vi "TestGeneralSyntax.vi"(8 "error in (no error)":errorcluster) -> (0 "error out":errorcluster)   [LabVIEW 2019]
uses:
  <vilib>/addons/_JKI Toolkits/Caraya/classes/Test/Test.lvclass
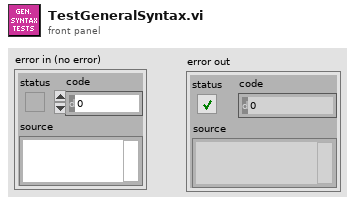
[diagram p1: front panel]
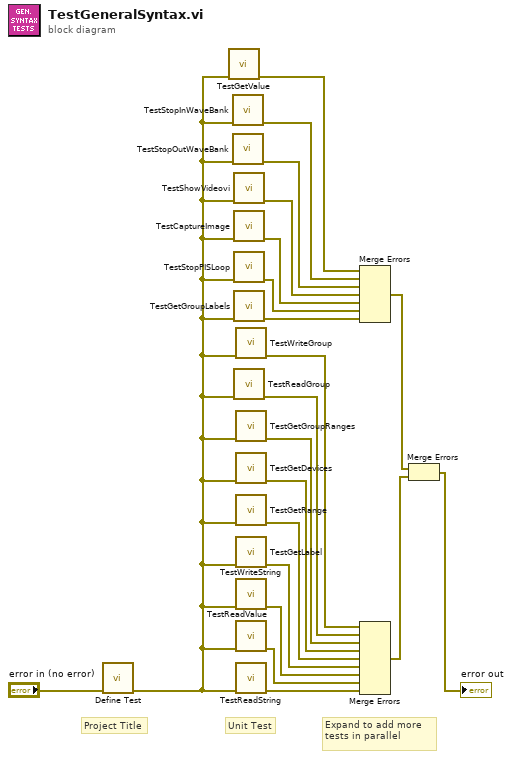
[diagram p0: block diagram]
diagram:
  # "Expand to add more tests in parallel"
  # "Unit Test"
  # "Project Title"
  n1 = call <vilib>:"Define Test.vi"("error in (no error)"="error in (no error)") -> ("error out"=w1:errorcluster)  [unwired: 10 in]
  n2 = call "TestGetValue.vi"("error in (no error)"=w1) -> ("error out"=w2:errorcluster)  [unwired: 10 in]
  n3 = call "TestStopInWaveBank.vi"("error in (no error)"=w1) -> ("error out"=w3:errorcluster)  [unwired: 10 in]
  n4 = call "TestStopOutWaveBank.vi"("error in (no error)"=w1) -> ("error out"=w4:errorcluster)  [unwired: 10 in]
  n5 = call "TestShowVideovi.vi"("error in (no error)"=w1) -> ("error out"=w5:errorcluster)  [unwired: 10 in]
  n6 = call "TestCaptureImage.vi"("error in (no error)"=w1) -> ("error out"=w6:errorcluster)  [unwired: 10 in]
  n7 = call "TestStopPISLoop.vi"("error in (no error)"=w1) -> ("error out"=w7:errorcluster)  [unwired: 10 in]
  n8 = call "TestGetGroupLabels.vi"("error in (no error)"=w1) -> ("error out"=w9:errorcluster)  [unwired: 10 in]
  n9 = call "TestReadGroup.vi"("error in (no error)"=w1) -> ("error out"=w13:errorcluster)  [unwired: 10 in]
  n10 = call "TestWriteGroup.vi"("error in (no error)"=w1) -> ("error out"=w12:errorcluster)  [unwired: 10 in]
  n11 = call "TestGetGroupRanges.vi"("error in (no error)"=w1) -> ("error out"=w14:errorcluster)  [unwired: 10 in]
  n12 = call "TestGetDevices.vi"("error in (no error)"=w1) -> ("error out"=w15:errorcluster)  [unwired: 10 in]
  n13 = call "TestGetRange.vi"("error in (no error)"=w1) -> ("error out"=w16:errorcluster)  [unwired: 10 in]
  n14 = call "TestGetLabel.vi"("error in (no error)"=w1) -> ("error out"=w17:errorcluster)  [unwired: 10 in]
  n15 = call "TestWriteString.vi"("error in (no error)"=w1) -> ("error out"=w18:errorcluster)  [unwired: 10 in]
  n16 = call "TestReadValue.vi"("error in (no error)"=w1) -> ("error out"=w19:errorcluster)  [unwired: 10 in]
  n17 = call "TestReadString.vi"("error in (no error)"=w1) -> ("error out"=w20:errorcluster)  [unwired: 10 in]
  n18 = Merge Errors(w2, w3, w4, w5, w6, w7, w9) -> (w10:errorcluster)
  n19 = Merge Errors(w12, w13, w14, w15, w16, w17, w18, w19, w20) -> (w11:errorcluster)
  n20 = Merge Errors(w10, w11) -> (→"error out":errorcluster)
